vi "AO SCTR Engine.vi"(0 "Unique Notifier Name":string, 11 "AO PFI Lines":string[](array[string])) -> ()   [LabVIEW 2016]
uses:
  AO SCTR Type Defs/AO SCTR Notifier Type.ctl
  AO SCTR Type Defs/AO SCTR Actions.ctl
  <vilib>/DAQmx/write.llb/DAQmx Write (Analog DBL 1Chan 1Samp).vi
  <vilib>/Analysis/1siggen.llb/Ramp Pattern by Samples.vi
  <vilib>/DAQmx/write.llb/DAQmx Write (Analog 1D DBL 1Chan NSamp).vi
  <vilib>/DAQmx/create/channels.llb/DAQmx Create Channel (AO-Voltage-Basic).vi
  <vilib>/DAQmx/miscellaneous.llb/DAQmx Fill In Error Info.vi
  <vilib>/DAQmx/configure/timing.llb/DAQmx Timing (Sample Clock).vi
  <resource>/objmgr/daqmx.rc
  <vilib>/Analysis/NI_AALBase.lvlib
panel:
  in  "Disable Input":bool
  out "Running":bool
  in  "Load":bool
  in  "Save":bool
  in  "Quit":bool
  in  "Waveform Settings":T1={"Actions"=enum."Stop at Offset", "Offset (V)"=-0.61, "Amplititude (V)"=0.524, "Samples Per Channel"=2280, "Start Delay (ms)"=20.0, "Running?"=FALSE} {"Amplititude (V)" format="%#_13g"; "Offset (V)" format="%#_13g"; "Start Delay (ms)" format="%#_13g"}
  out "Waveform Graph":dbl[](graph)
  out "Actual Sample Rate":dbl=10000.0 format="%0.2f"
  # "AO Line Example: Dev1/ao1\nPFI Line Example: /Dev1/PFI0"
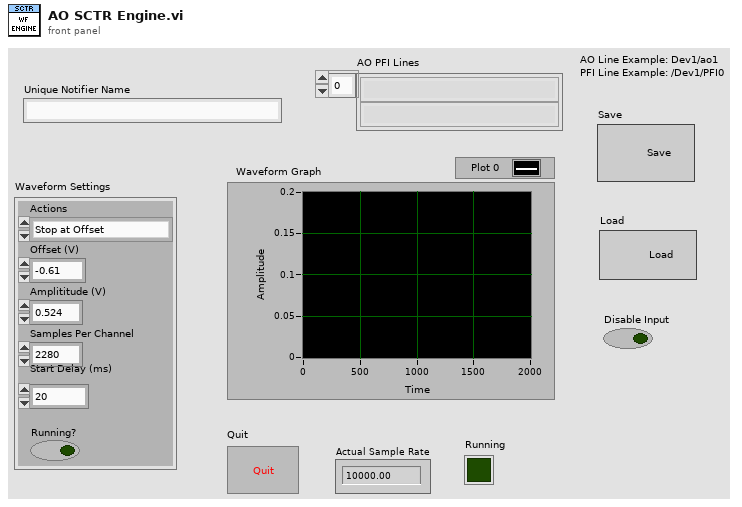
[diagram p1: front panel]
types:
  T1 = typedef "AO SCTR Notifier Type.ctl" = cluster{"Actions":T2, "Offset (V)":dbl, "Amplititude (V)":dbl, "Samples Per Channel":i32, "Start Delay (ms)":dbl, "Running?":bool}
  T2 = typedef "AO SCTR Actions.ctl" = enum16{"Stop at Offset", "Update and Run", "Quit"}
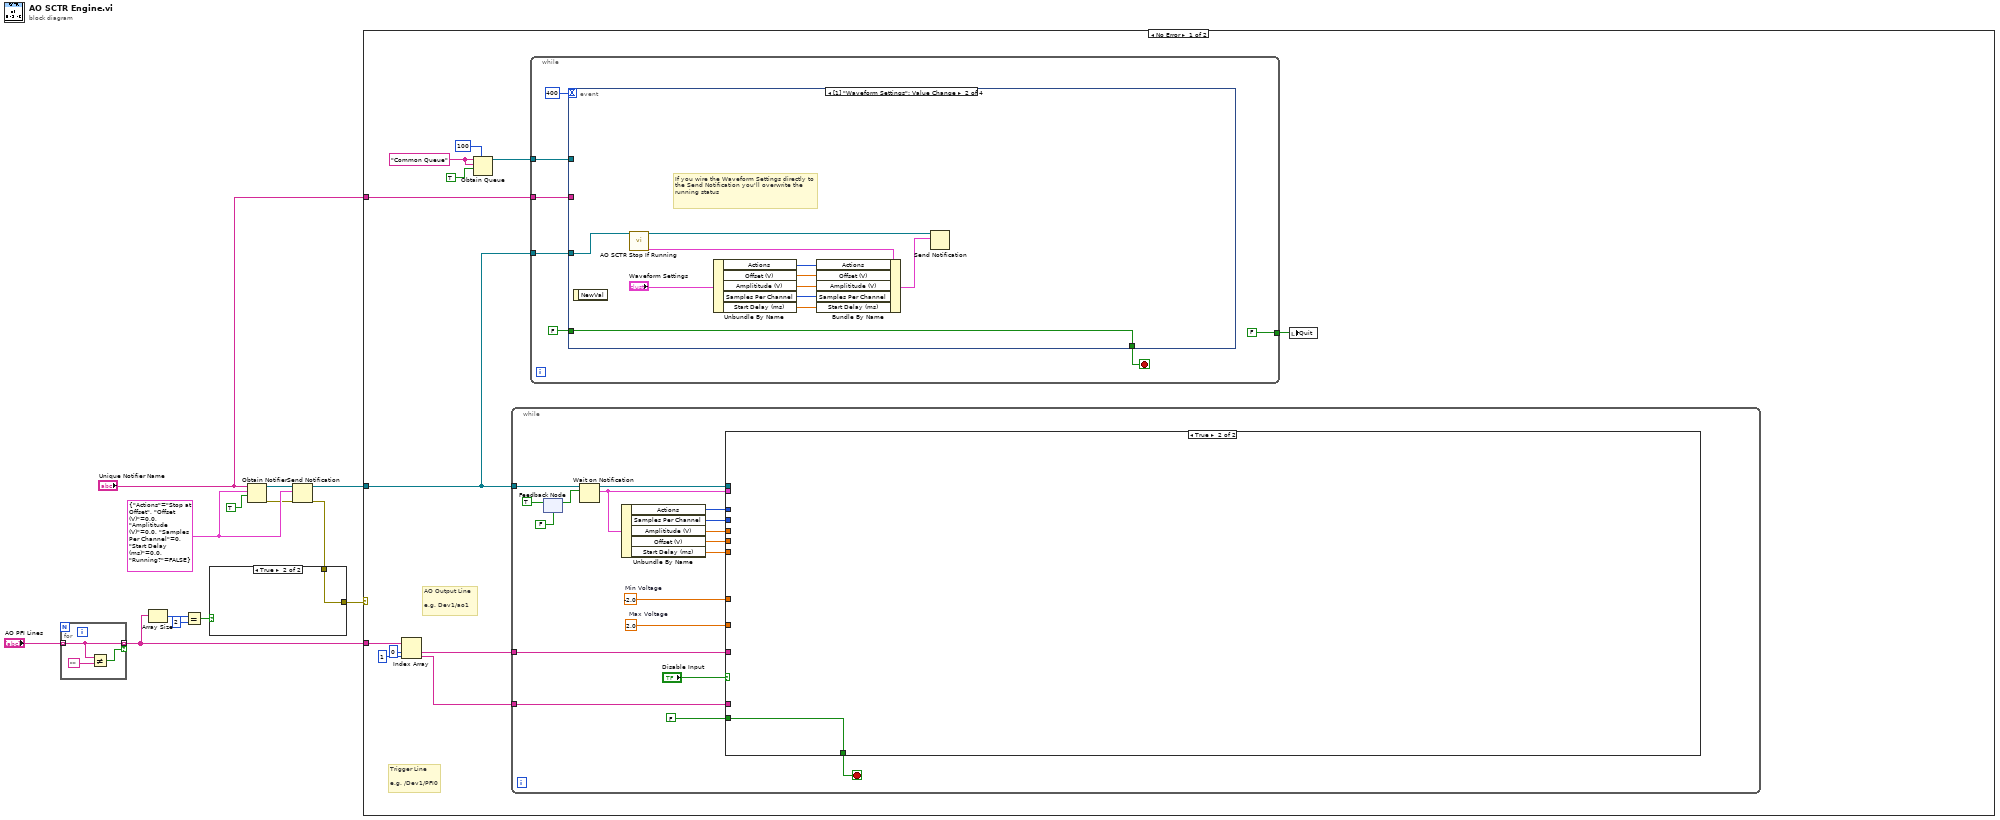
[diagram p0: block diagram]
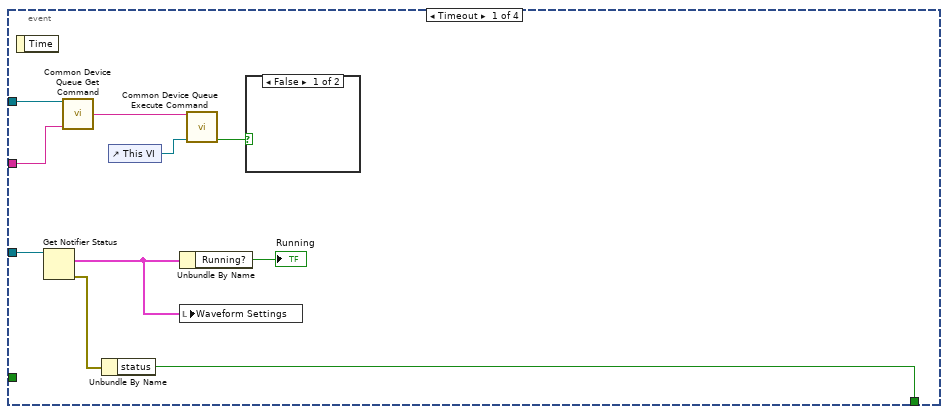
[diagram p2: hidden frame]
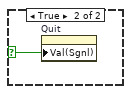
[diagram p3: hidden frame]
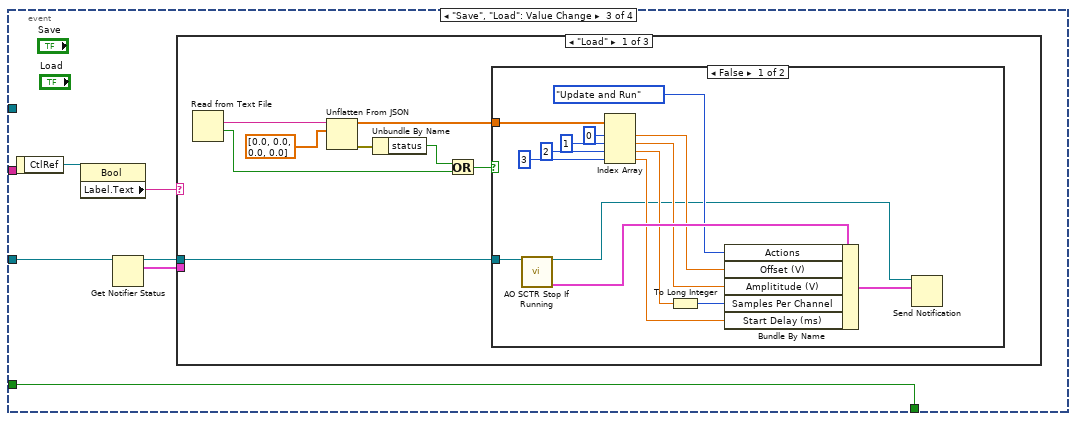
[diagram p4: hidden frame]
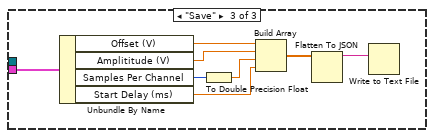
[diagram p7: hidden frame]
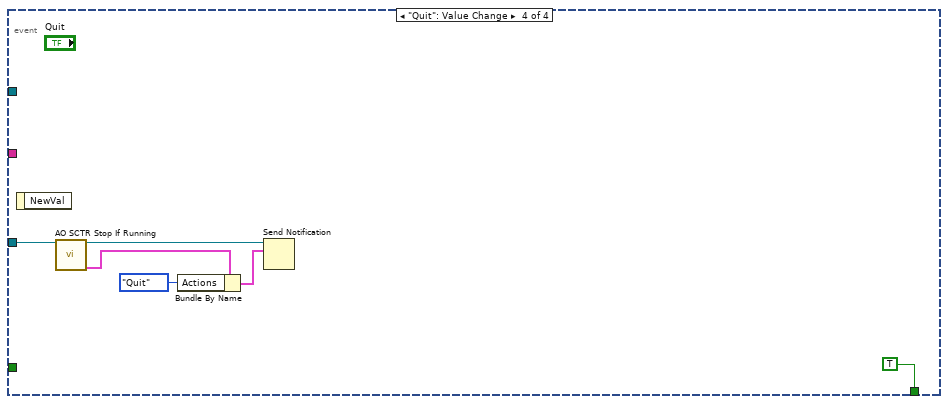
[diagram p8: hidden frame]
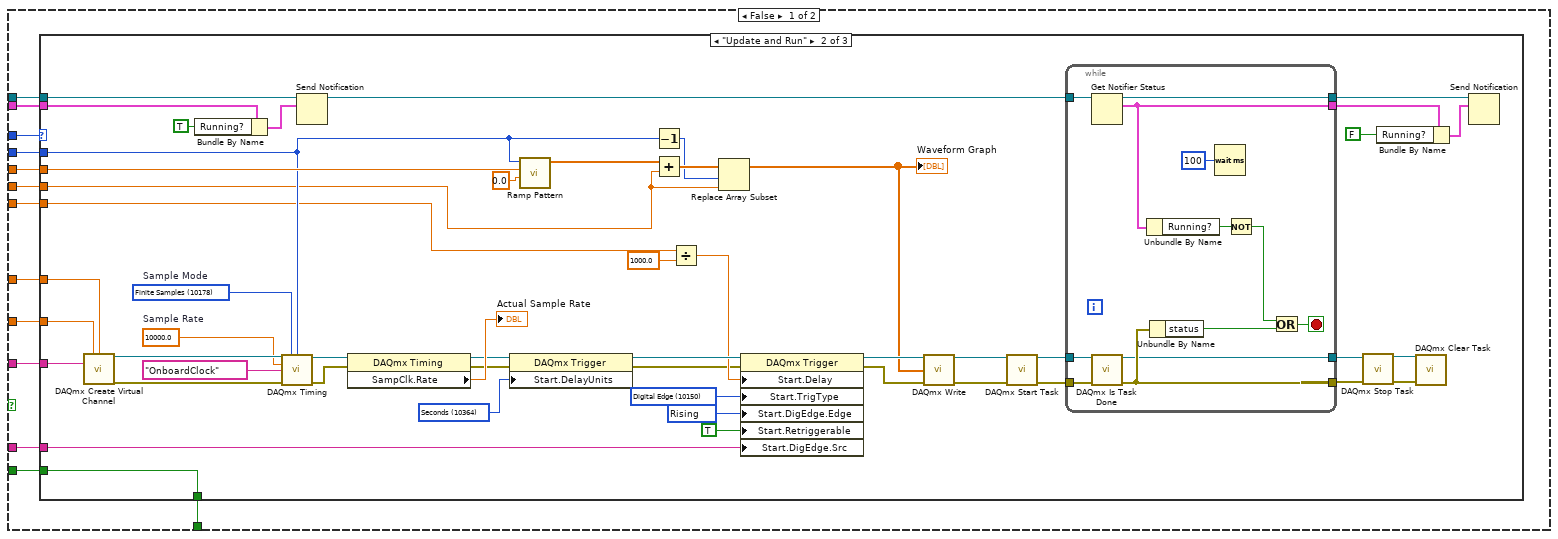
[diagram p9: hidden frame]
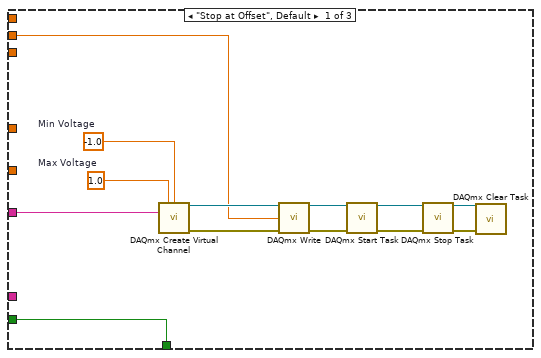
[diagram p10: hidden frame]
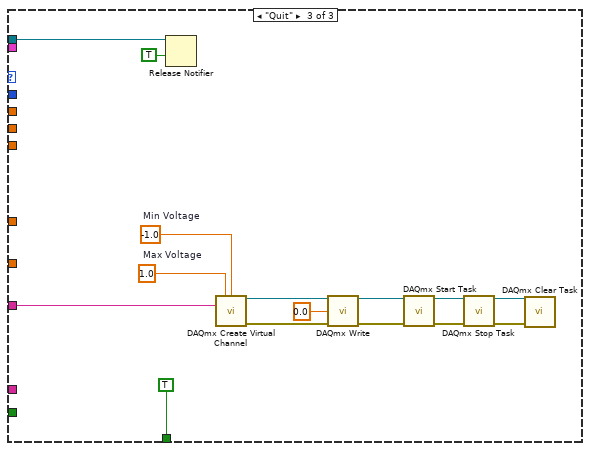
[diagram p11: hidden frame]
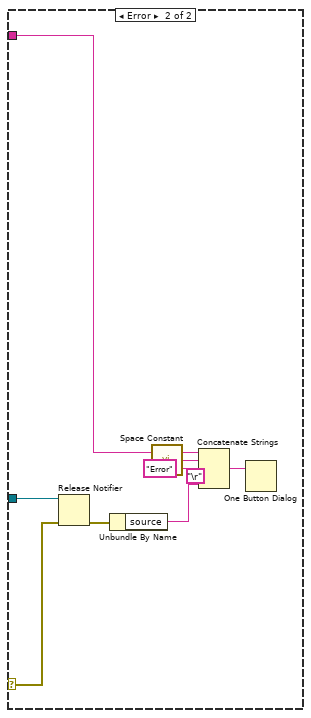
[diagram p12: hidden frame]
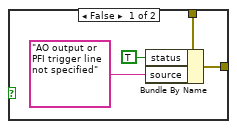
[diagram p13: hidden frame]
diagram:
  w8 = T1 {"Actions"=enum."Stop at Offset", "Offset (V)"=0.0, "Amplititude (V)"=0.0, "Samples Per Channel"=0, "Start Delay (ms)"=0.0, "Running?"=FALSE} ("Waveform Settings 2")
  n1 = for {
    tunnel: "AO PFI Lines" -> [w15] mode=indexing
    tunnel: [w15] -> w6 mode=indexing if=w14
    n2 = Not Equal?(x=w15, y="") -> (x != y?=w14:bool)
  }
  n3 = Array Size(array=w6) -> (size(s)=w5:i32)
  n4 = Equal?(x=w5, y=2) -> (x = y?=w3:bool)
  n5 = Obtain Notifier(name (unnamed)="Unique Notifier Name", notification data type=w8, create if not found? (T)=TRUE) -> (notifier out=w10:refnum<notifier>, error out=w7:errorcluster)  [unwired: 1 in, 1 out]
  n6 = Send Notification(notification=w8, notifier=w10, error in (no error)=w7) -> (notifier out=w9:refnum<notifier>, error out=w2:errorcluster)
  n7 = case shown="True" w3 {
    tunnel: w2 -> [w20 w21]
    tunnel: [w19 w21] -> w1
    frame False {
      n8 = Bundle By Name(cluster=w20, "status"=TRUE, "source"="AO output or PFI trigger line not specified") -> (w19:errorcluster)
    }
    frame True {
    }
  }
  n9 = case shown="No Error" w1 {
    selector: w1 -> [_ w236]
    tunnel: "Unique Notifier Name" -> [w28 w234]
    tunnel: w9 -> [w23 w237]
    tunnel: w6 -> [w22 _]
    frame No Error {
      w33 = "Common Queue" ("Unique Notifier Name")
      # "Trigger Line\n\ne.g. /Dev1/PFI0"
      # "AO Output Line\n\ne.g. Dev1/ao1"
      n10 = Index Array(array=w22, index #1=0 ("index"), index #2=1 ("index")) -> (element #1=w25:string, element #2=w24:string)
      n11 = Obtain Queue(max queue size (-1, unlimited)=100, name (unnamed)=w33, element data type=w33, create if not found? (T)=TRUE) -> (queue out=w29:refnum<queue>)  [unwired: 1 in, 2 out]
      n12 = while {
        tunnel: w23 -> [w107]
        tunnel: w25 -> [w115]
        tunnel: w24 -> [w114]
        stop <- w116 stop-if-true
        w109 = 2.0  # Max Voltage
        w110 = -2.0  # Min Voltage
        n13 = feedback-in #1(TRUE ("ignore previous (F)")) -> ()
        n14 = feedback #1(FALSE ("ignore previous (F)")) -> (w111:bool)
        n15 = Wait on Notification(notifier=w107, ignore previous (F)=w111) -> (notifier out=w118:refnum<notifier>, notification=w117:T1)  [unwired: 2 in, 2 out]
        n16 = Unbundle By Name(w117) -> ("Actions"=w119:T2, "Samples Per Channel"=w121:i32, "Amplititude (V)"=w123:dbl, "Offset (V)"=w120:dbl, "Start Delay (ms)"=w122:dbl)
        n17 = case shown="True" "Disable Input" {
          tunnel: w123 -> [w136 _]
          tunnel: w122 -> [w135 _]
          tunnel: w121 -> [w134 _]
          tunnel: w120 -> [w133 _]
          tunnel: w119 -> [w132 _]
          tunnel: w118 -> [w131 _]
          tunnel: w117 -> [w130 _]
          tunnel: [w129 w228] -> w116
          tunnel: w115 -> [w128 _]
          tunnel: w114 -> [w127 _]
          tunnel: w110 -> [w126 _]
          tunnel: w109 -> [w125 _]
          tunnel: FALSE -> [w124 w228]
          frame False {
            n18 = case shown="\"Update and Run\"" w132 {
              tunnel: w136 -> [_ w174 _]
              tunnel: w135 -> [_ w154 _]
              tunnel: w134 -> [_ w173 _]
              tunnel: w133 -> [w139 w172 _]
              tunnel: w131 -> [_ w171 w225]
              tunnel: w130 -> [_ w169 _]
              tunnel: [w138 w163 TRUE] -> w129
              tunnel: w128 -> [w137 w166 w213]
              tunnel: w127 -> [_ w158 _]
              tunnel: w126 -> [_ w165 _]
              tunnel: w125 -> [_ w164 _]
              tunnel: w124 -> [w138 w163 _]
              frame "Stop at Offset", Default {
                w141 = 1.0  # Max Voltage
                w140 = -1.0  # Min Voltage
                n19 = call-poly <vilib>:"DAQmx Create Virtual Channel.vi"("maximum value"=w141, "minimum value"=w140, "physical channels"=w137) -> ("task out"=w142:refnum<k21>, "error out"=w147:errorcluster)  [unwired: 11 in]
                n20 = call-poly <vilib>:"DAQmx Write.vi"("task/channels in"=w142, "data"=w139, "error in"=w147) -> ("task out"=w143:refnum<k21>, "error out"=w148:errorcluster)  [unwired: 10 in, 1 out]
                n21 = call <vilib>:"DAQmx Start Task.vi"("task/channels in"=w143, "error in"=w148) -> ("task out"=w145:refnum<k21>, "error out"=w149:errorcluster)  [unwired: 12 in]
                n22 = call <vilib>:"DAQmx Stop Task.vi"("task/channels in"=w145, "error in"=w149) -> ("task out"=w146:refnum<k21>, "error out"=w144:errorcluster)  [unwired: 12 in]
                n23 = call <vilib>:"DAQmx Clear Task.vi"("task in"=w146, "error in"=w144) -> ()  [unwired: 13 in, 1 out]
              }
              frame "Update and Run" {
                w157 = 10364 items=["Sample Clock Periods"=10286, "Seconds"=10364, "Ticks"=10304] ("Start.DelayUnits")
                w193 = 10000.0  # Sample Rate
                w185 = 10280 items=["Rising"=10280, "Falling"=10171] ("Start.DigEdge.Edge")
                w175 = 10150 items=["Analog Edge"=10099, "Digital Edge"=10150, "Digital Pattern"=10398, "Analog Window"=10103, "None"=10230] ("Start.TrigType")
                w199 = 10178 items=["Finite Samples"=10178, "Continuous Samples"=10123, "Hardware Timed Single Point"=12522]  # Sample Mode
                n24 = call-poly <vilib>:"DAQmx Create Virtual Channel.vi"("maximum value"=w164, "minimum value"=w165, "physical channels"=w166) -> ("task out"=w197:refnum<k21>, "error out"=w198:errorcluster)  [unwired: 11 in]
                n25 = Bundle By Name(cluster=w169, "Running?"=TRUE ("Running")) -> (w167:T1)
                n26 = call-poly <vilib>:"DAQmx Timing.vi"("task/channels in"=w197, "sample mode"=w199, "samples per channel"=w173, "rate"=w193, "source"=tag "OnboardClock" ("Sample Clock Source"), "error in"=w198) -> ("task out"=w183:refnum<k21>, "error out"=w200:errorcluster)  [unwired: 8 in]
                n27 = Send Notification(notification=w167, notifier=w171) -> (notifier out=w170:refnum<notifier>)  [unwired: 1 in, 1 out]
                n28 = property class="DAQmx Timing"(reference=w183, error in=w200) -> (reference out=w156:refnum<k21>, error out=w150:errorcluster, "SampClk.Rate"=→"Actual Sample Rate":dbl)
                n29 = property class="DAQmx Trigger"(reference=w156, error in=w150, "Start.DelayUnits"=w157) -> (reference out=w155:refnum<k21>, error out=w151:errorcluster)
                n30 = call-poly <vilib>:"Ramp Pattern.vi"("start"=0.0, "end"=w174, "samples"=w173) -> ("Ramp Pattern"=w179:dbl[])  [unwired: 7 in, 1 out]
                n31 = Decrement(x=w173) -> (x-1=w177:i32)
                n32 = Add(x=w179, y=w172) -> (x+y=w178:dbl[])
                n33 = Divide(x=w154, y=1000.0) -> (x/y=w153:dbl)
                n34 = Replace Array Subset(array=w178, new element=w172, index=w177) -> (w176:dbl[])
                "Waveform Graph" <- w176
                n35 = property class="DAQmx Trigger"(reference=w155, error in=w151, "Start.Delay"=w153, "Start.TrigType"=w175, "Start.DigEdge.Edge"=w185, "Start.Retriggerable"=TRUE, "Start.DigEdge.Src"=w158) -> (reference out=w186:refnum<k21>, error out=w180:errorcluster)
                n36 = call-poly <vilib>:"DAQmx Write.vi"("task/channels in"=w186, "data"=w176, "error in"=w180) -> ("task out"=w192:refnum<k21>, "error out"=w191:errorcluster)  [unwired: 10 in, 1 out]
                n37 = call <vilib>:"DAQmx Start Task.vi"("task/channels in"=w192, "error in"=w191) -> ("task out"=w196:refnum<k21>, "error out"=w195:errorcluster)  [unwired: 12 in]
                n38 = while {
                  tunnel: w196 -> [w212]
                  tunnel: w195 -> [w211]
                  tunnel: [w210] -> w187
                  tunnel: [w209] -> w188
                  tunnel: w170 -> [w206]
                  tunnel: [w204] -> w162
                  tunnel: [w203] -> w159
                  stop <- w208 stop-if-true
                  n39 = Get Notifier Status(notifier=w206) -> (notifier out=w204:refnum<notifier>, current notification=w203:T1)  [unwired: 1 in, 3 out]
                  n40 = call <vilib>:"DAQmx Is Task Done.vi"("task/channels in"=w212, "error in"=w211) -> ("task out"=w209:refnum<k21>, "error out"=w210:errorcluster)  [unwired: 11 in, 1 out]
                  n41 = Unbundle By Name(w203) -> ("Running?"=w205:bool)
                  n42 = Unbundle By Name(w210) -> ("status"=w207:bool)
                  n43 = Wait (ms)(milliseconds to wait=u32 100) -> ()  [unwired: 1 out]
                  n44 = Not(x=w205) -> (.not. x?=w202:bool)
                  n45 = Or(x=w202, y=w207) -> (x .or. y?=w208:bool)
                }
                n46 = call <vilib>:"DAQmx Stop Task.vi"("task/channels in"=w188, "error in"=w187) -> ("task out"=w190:refnum<k21>, "error out"=w189:errorcluster)  [unwired: 12 in]
                n47 = Bundle By Name(cluster=w159, "Running?"=FALSE ("Running")) -> (w160:T1)
                n48 = call <vilib>:"DAQmx Clear Task.vi"("task in"=w190, "error in"=w189) -> ()  [unwired: 13 in, 1 out]
                n49 = Send Notification(notification=w160, notifier=w162) -> ()  [unwired: 1 in, 2 out]
              }
              frame "Quit" {
                w216 = 1.0  # Max Voltage
                w215 = -1.0  # Min Voltage
                n50 = Release Notifier(notifier=w225, force destroy? (F)=TRUE) -> ()  [unwired: 1 in, 3 out]
                n51 = call-poly <vilib>:"DAQmx Create Virtual Channel.vi"("maximum value"=w216, "minimum value"=w215, "physical channels"=w213) -> ("task out"=w217:refnum<k21>, "error out"=w222:errorcluster)  [unwired: 11 in]
                n52 = call-poly <vilib>:"DAQmx Write.vi"("task/channels in"=w217, "data"=0.0, "error in"=w222) -> ("task out"=w218:refnum<k21>, "error out"=w223:errorcluster)  [unwired: 10 in, 1 out]
                n53 = call <vilib>:"DAQmx Start Task.vi"("task/channels in"=w218, "error in"=w223) -> ("task out"=w220:refnum<k21>, "error out"=w224:errorcluster)  [unwired: 12 in]
                n54 = call <vilib>:"DAQmx Stop Task.vi"("task/channels in"=w220, "error in"=w224) -> ("task out"=w221:refnum<k21>, "error out"=w219:errorcluster)  [unwired: 12 in]
                n55 = call <vilib>:"DAQmx Clear Task.vi"("task in"=w221, "error in"=w219) -> ()  [unwired: 13 in, 1 out]
              }
            }
          }
          frame True {
          }
        }
      }
      n56 = while {
        tunnel: w23 -> [w40]
        tunnel: [FALSE] -> w30
        tunnel: w29 -> [w36]
        tunnel: w28 -> [w35]
        stop <- w38 stop-if-true
        n57 = event shown="[1] \"Waveform Settings\": Value Change" {
          selector: _ -> [_ _ _ _]
          dyn-events: _ -> [_ _ _ _]
          timeout: 400 -> [_ _ _ _]
          tunnel: w40 -> [w50 w61 w66 w102]
          tunnel: [w48 w62 w63 TRUE ("status")] -> w38
          tunnel: w36 -> [w44 _ _ _]
          tunnel: w35 -> [w43 _ _ _]
          tunnel: FALSE ("status") -> [_ w62 w63 _]
          event Timeout {
            n58 = event-data() -> ()  [unwired: 1 in, 1 out]
            n59 = Get Notifier Status(notifier=w50) -> (current notification=w41:T1, error out=w49:errorcluster)  [unwired: 1 in, 3 out]
            n60 = call "Common Device Queue Get Command.vi"("Common Queue"=w44, "Notifier Name"=w43) -> ("Command"=w46:string)  [unwired: 12 in, 1 out]
            n61 = Unbundle By Name(w49) -> ("status"=w48:bool)
            n62 = control-ref of="This VI"() -> (w45:refnum<vi>)
            n63 = Unbundle By Name(w41) -> ("Running?"=→"Running":bool)
            n64 = local write "Waveform Settings"(w41) -> ()
            n65 = call "Common Device Queue Execute Command.vi"("Common Command"=w46, "VI Refnum"=w45) -> ("Quit?"=w47:bool)  [unwired: 12 in, 1 out]
            n66 = case shown="False" w47 {
              selector: w47 -> [_ w51]
              frame False {
              }
              frame True {
                n67 = property on="Quit" class="Bool (strict)"("Val(Sgnl)"=w51) -> ()  [unwired: 2 in, 2 out]
              }
            }
          }
          event Value Change {
            # "If you wire the Waveform Settings directly to the Send Notification you'll overwrite the running status"
            n68 = event-data() -> ()  [unwired: 1 in, 1 out]
            n69 = call "AO SCTR Stop If Running.vi"("AO SCTR Notifier"=w61) -> ("AO SCTR Notifier (Dup)"=w60:refnum<notifier>, "Latest Notification"=w59:T1)  [unwired: 13 in]
            n70 = Unbundle By Name("Waveform Settings") -> ("Actions"=w56:T2, "Offset (V)"=w55:dbl, "Amplititude (V)"=w54:dbl, "Samples Per Channel"=w53:i32, "Start Delay (ms)"=w52:dbl)
            n71 = Bundle By Name(cluster=w59, "Actions"=w56, "Offset (V)"=w55, "Amplititude (V)"=w54, "Samples Per Channel"=w53, "Start Delay (ms)"=w52) -> (w58:T1)
            n72 = Send Notification(notification=w58, notifier=w60) -> ()  [unwired: 1 in, 2 out]
          }
          event "Save", "Load": Value Change {
            n73 = event-data() -> ("CtlRef"=w68:refnum<vi>)  [unwired: 1 in]
            n74 = property class="Bool"(reference=w68) -> ("Label.Text"=w67:string)  [unwired: 1 in, 2 out]
            n75 = Get Notifier Status(notifier=w66) -> (notifier out=w64:refnum<notifier>, current notification=w65:T1)  [unwired: 1 in, 3 out]
            n76 = case shown="\"Load\"" w67 {
              tunnel: w65 -> [_ _ w99]
              tunnel: w64 -> [w70 _ _]
              frame "Load" {
                n77 = Read from Text File() -> (text=w76:string, cancelled=w72:bool)  [unwired: 4 in, 2 out]
                n78 = Unflatten From JSON(JSON string=w76, type and defaults=dbl[] [0.0, 0.0, 0.0, 0.0]) -> (value=w69:dbl[], error out=w74:errorcluster)  [unwired: 5 in]
                n79 = Unbundle By Name(w74) -> ("status"=w73:bool)
                n80 = Or(x=w73, y=w72) -> (x .or. y?=w71:bool)
                n81 = case shown="False" w71 {
                  tunnel: w70 -> [w91 _]
                  tunnel: w69 -> [w88 _]
                  frame False {
                    n82 = call "AO SCTR Stop If Running.vi"("AO SCTR Notifier"=w91) -> ("AO SCTR Notifier (Dup)"=w78:refnum<notifier>, "Latest Notification"=w90:T1)  [unwired: 13 in]
                    n83 = Index Array(array=w88, index #1=0 ("index"), index #2=1 ("index"), index #3=2 ("index"), index #4=3 ("index")) -> (element #1=w79:dbl, element #2=w80:dbl, element #3=w82:dbl, element #4=w83:dbl)
                    n84 = To Long Integer(number=w82) -> (32bit integer=w81:i32)
                    n85 = Bundle By Name(cluster=w90, "Actions"=AO_SCTR_Actions."Update and Run", "Offset (V)"=w79, "Amplititude (V)"=w80, "Samples Per Channel"=w81, "Start Delay (ms)"=w83) -> (w77:T1)
                    n86 = Send Notification(notification=w77, notifier=w78) -> ()  [unwired: 1 in, 2 out]
                  }
                  frame True {
                  }
                }
              }
              frame Default {
              }
              frame "Save" {
                n87 = Unbundle By Name(w99) -> ("Offset (V)"=w98:dbl, "Amplititude (V)"=w95:dbl, "Samples Per Channel"=w96:i32, "Start Delay (ms)"=w97:dbl)
                n88 = To Double Precision Float(number=w96) -> (double precision float=w94:dbl)
                n89 = Build Array(w98, w95, w94, w97) -> (w93:dbl[])
                n90 = Flatten To JSON(anything=w93) -> (JSON string=w92:string)  [unwired: 2 in, 1 out]
                n91 = Write to Text File(text=w92) -> ()  [unwired: 3 in, 3 out]
              }
            }
          }
          event "Quit": Value Change {
            n92 = event-data() -> ()  [unwired: 1 in, 1 out]
            n93 = call "AO SCTR Stop If Running.vi"("AO SCTR Notifier"=w102) -> ("AO SCTR Notifier (Dup)"=w101:refnum<notifier>, "Latest Notification"=w100:T1)  [unwired: 13 in]
            n94 = Bundle By Name(cluster=w100, "Actions"=AO_SCTR_Actions."Quit") -> (w104:T1)
            n95 = Send Notification(notification=w104, notifier=w101) -> ()  [unwired: 1 in, 2 out]
          }
        }
      }
      n96 = local write "Quit"(w30) -> ()
    }
    frame Error {
      n97 = Release Notifier(notifier=w237, error in (no error)=w236) -> (error out=w230:errorcluster)  [unwired: 1 in, 2 out]
      n98 = Unbundle By Name(w230) -> ("source"=w229:string)
      n99 = call <vilib>:"Space Constant.vi"() -> ("String"=w233:string)
      n100 = Concatenate Strings(w234, w233, "Error" ("string"), "\r", w229) -> (w235:string)
      n101 = One Button Dialog(message=w235) -> ()  [unwired: 1 in, 1 out]
    }
  }
